vi "LinearSystemId_IdentifyVelocitySystem.vi"(10 "kA":dbl, 11 "kV":dbl) -> (0 "Size Coerced":bool, 3 "Linearsystem":T1)   [LabVIEW 2019, in "Trajectory_Library.lvlib"]
doc: "Identify a velocity system from it's kV (volts/(unit/sec)) and kA (volts/(unit/sec^2). These constants cam be found using frc-characterization. The states of the system are [velocity], inputs are [voltage], and outputs are [velocity].\n\nThe distance unit you choose MUST be an SI unit (i.e. meters or radians). You can use the Util.Units subVI for converting between unit types.\n\nInputs:\n - kV -- The velocity gain, in volts per (units per second)\n - kA -- The acceleration gain, in volts per (units per second squared)\n\nOutputs:\n - LinearSystem -- A LinearSystem representing the given characterized constants.\n - SizeCoerced -- A value of TRUE indicates an unexpected error occured.\n\nAdditional information:\n See https://github.com/wpilibsuite/frc-characterization"
uses:
  Trajectory_Library.lvlib
  TypeDef/LINEAR_SYSTEM.ctl
  <vilib>/Analysis/Matrix/Datatypes/RealMatrix.ctl
  <vilib>/Analysis/Matrix/NI_Matrix.lvlib
panel:
  # "<States,States>"
  # "<States,Inputs>"
  # "<Outputs,States>"
  # "<Outputs,Inputs>"
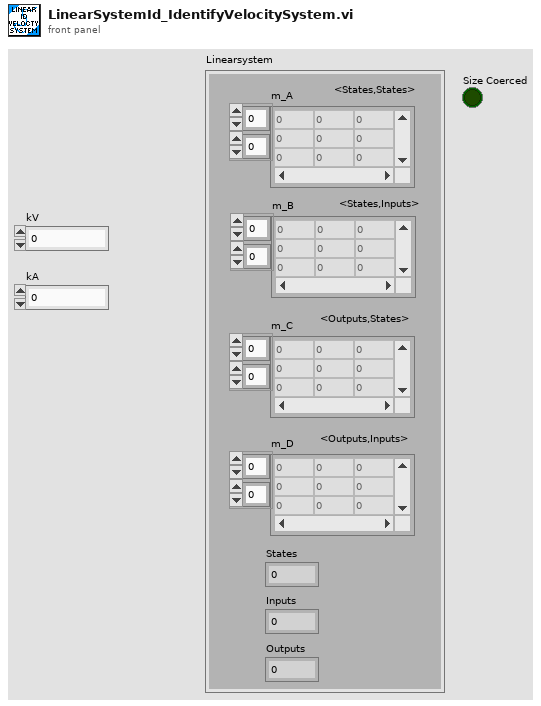
[diagram p1: front panel]
types:
  T1 = typedef "Trajectory_Library.lvlib/LINEAR_SYSTEM.ctl" = cluster{"m_A":T2, "m_B":T2, "m_C":T2, "m_D":T2, "States":i32, "Inputs":i32, "Outputs":i32}
  T2 = typedef "NI_Matrix.lvlib/RealMatrix.ctl" = dbl[][]
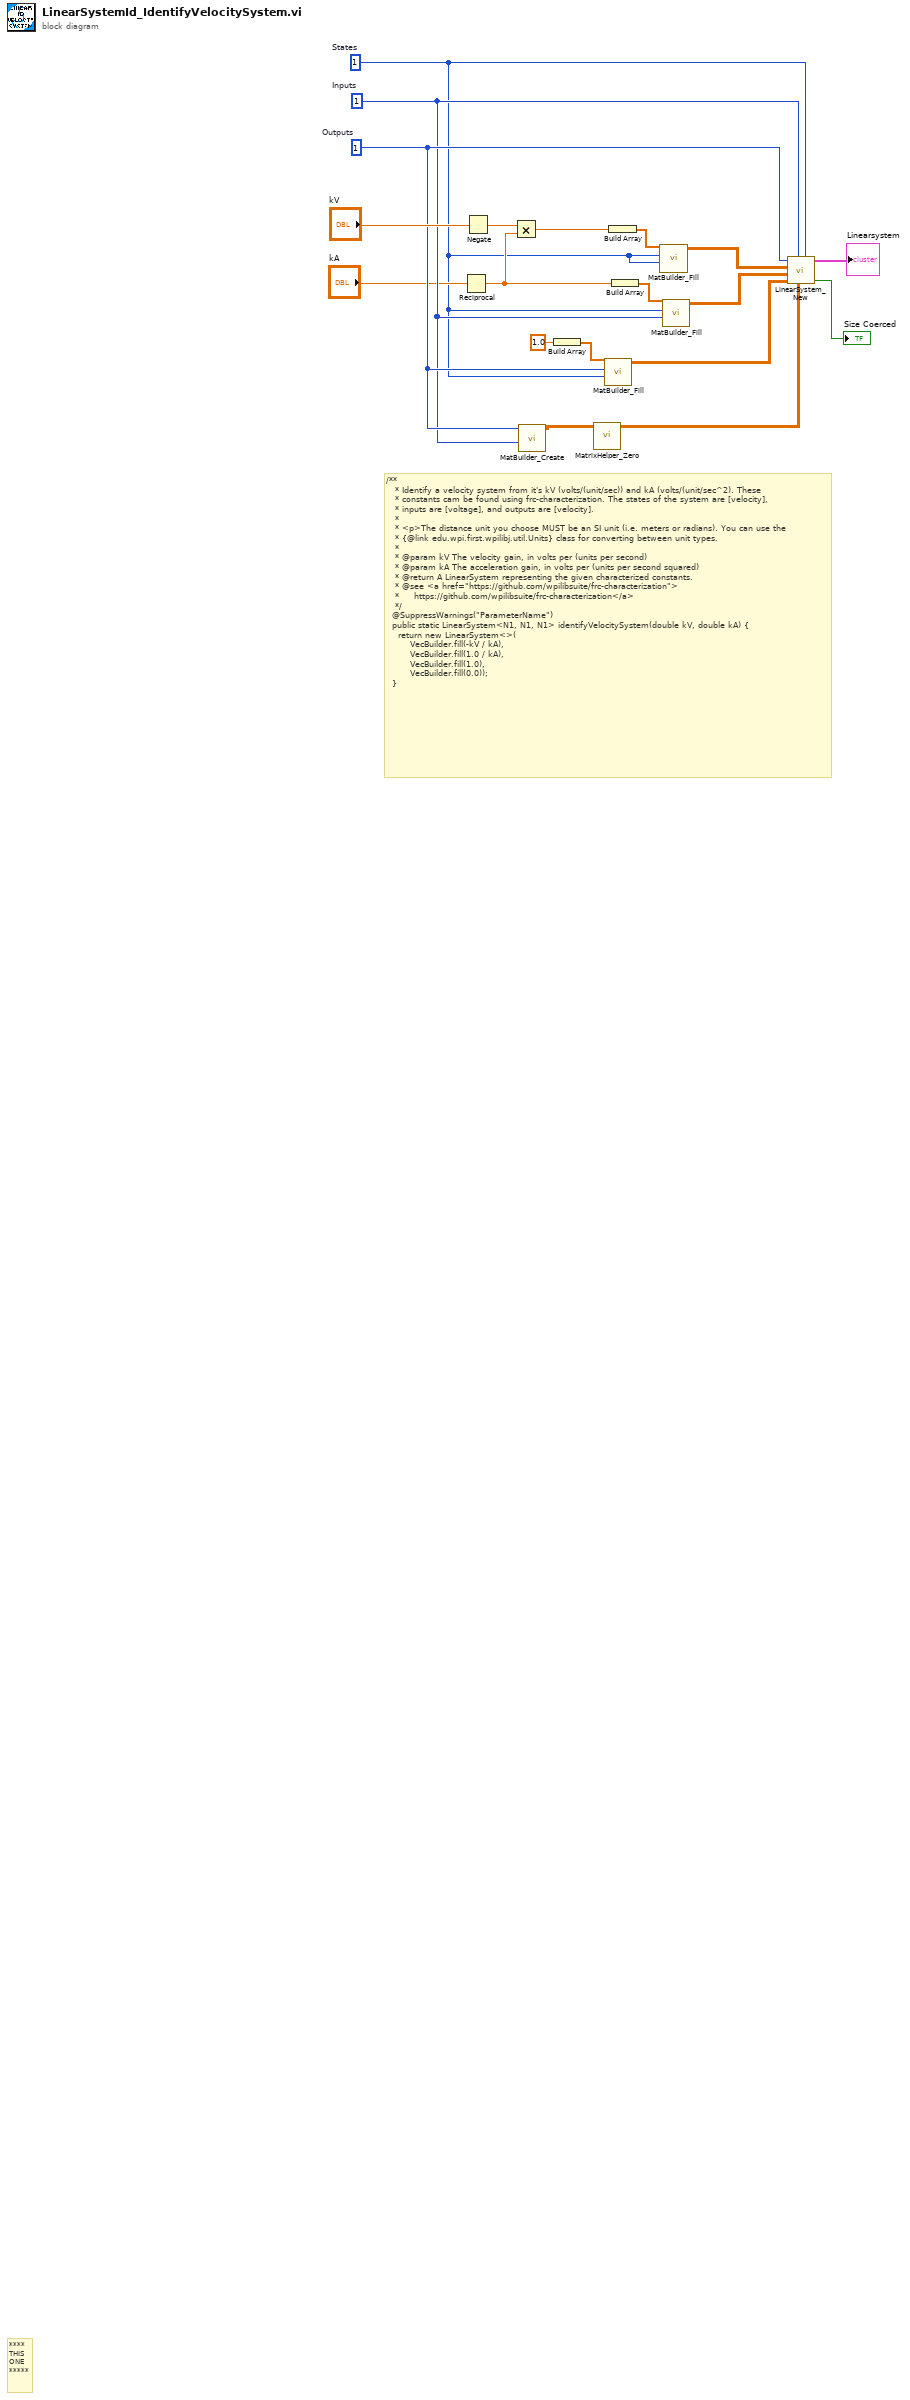
[diagram p0: block diagram]
diagram:
  w15 = 1  # Outputs
  w10 = 1  # Inputs
  w4 = 1  # States
  # "/**\n   * Identify a velocity system from it's kV (volts/(unit/sec)) and kA (volts/(unit/sec^2). These\n   * constants cam be found using frc-characterization. The states of the system are [velocity],\n   * inputs are [voltage], and outputs are [velocity].\n   *\n   * <p>The distance unit you choose MUST be an SI unit (i.e. meters or radians). You can use the\n   * {@link edu.wpi.first.wpilibj.util.Units} class for converting between unit types.\n   *\n   * @param kV The velocity gain, in volts per (units per second)\n   * @param kA The acceleration gain, in volts per (units per second squared)\n   * @return A LinearSystem representing the given characterized constants.\n   * @see <a href=\"https://github.com/wpilibsuite/frc-characterization\">\n   *     https://github.com/wpilibsuite/frc-characterization</a>\n   */\n  @SuppressWarnings(\"ParameterName\")\n  public static LinearSystem<N1, N1, N1> identifyVelocitySystem(double kV, double kA) {\n    return new LinearSystem<>(\n        VecBuilder.fill(-kV / kA),\n        VecBuilder.fill(1.0 / kA),\n        VecBuilder.fill(1.0),\n        VecBuilder.fill(0.0));\n  }"
  # "****\nTHIS\nONE\n*****"
  n1 = Reciprocal(x="kA") -> (1/x=w7:dbl)
  n2 = Negate(x="kV") -> (-x=w6:dbl)
  n3 = Multiply(x=w6, y=w7) -> (x*y=w3:dbl)
  n4 = call "MatBuilder_Create.vi"("Columns"=w10, "Rows"=w15) -> ("output matrix"=w17:T2)  [unwired: 9 in]
  n5 = Build Array(1.0 ("element")) -> (w13:dbl[])
  n6 = call "MatrixHelper_Zero.vi"("input matrix"=w17) -> ("output matrix"=w16:T2)  [unwired: 10 in]
  n7 = call "MatBuilder_Fill.vi"("Columns"=w4, "Rows"=w15, "Value List"=w13) -> ("output matrix"=w12:T2)  [unwired: 8 in]
  n8 = Build Array(w3) -> (w5:dbl[])
  n9 = Build Array(w7) -> (w11:dbl[])
  n10 = call "MatBuilder_Fill.vi"("Columns"=w4, "Rows"=w4, "Value List"=w5) -> ("output matrix"=w2:T2)  [unwired: 8 in]
  n11 = call "MatBuilder_Fill.vi"("Columns"=w10, "Rows"=w4, "Value List"=w11) -> ("output matrix"=w8:T2)  [unwired: 8 in]
  n12 = call "LinearSystem_New.vi"("States"=w4, "D"=w16, "Inputs"=w10, "C"=w12, "B"=w8, "A"=w2, "Outputs"=w15) -> ("Size Coerced"=→"Size Coerced":bool, "Linearsystem"=→"Linearsystem":T1)  [unwired: 3 in]
